vi "Format Spreadsheet Header.vi"(10 "Channel Settings":T1[](array[typedef])) -> (2 "Log file header":string)   [LabVIEW 2021, in "Logging.lvlib"]
doc: "Format a starting timestamp and column headings using the channel names from 'Channel Settings'."
uses:
  Logging.lvlib
  Acquisition/Channel Settings.ctl
  Acquisition/IO Device.ctl
  Acquisition/Sensor Type.ctl
  Acquisition/Acquisition.lvlib
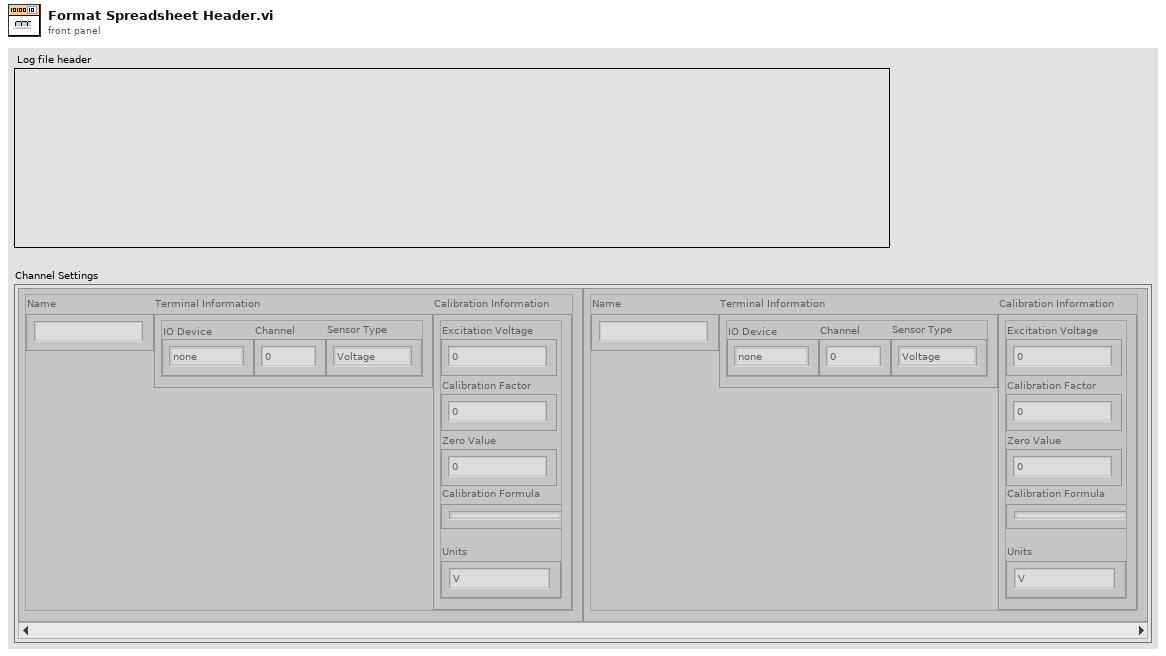
[diagram p1: front panel]
types:
  T1 = typedef "Acquisition.lvlib/Channel Settings.ctl" = cluster{"Name":string, "Terminal Information":cluster{"IO Device":T2, "Channel":i32, "Sensor Type":T3}, "Calibration Information":cluster{"Excitation Voltage":dbl, "Calibration Factor":dbl, "Zero Value":dbl, "Calibration Formula":string, "Units":string}}
  T2 = typedef "Acquisition.lvlib/IO Device.ctl" = enum16{"none", "9219", "9401"}
  T3 = typedef "Acquisition.lvlib/Sensor Type.ctl" = enum16{"Voltage", "Load", "Pressure", "Encoder"}
  T4 = cluster{"IO Device":T2, "Channel":i32, "Sensor Type":T3}
  T5 = cluster{"Excitation Voltage":dbl, "Calibration Factor":dbl, "Zero Value":dbl, "Calibration Formula":string, "Units":string}
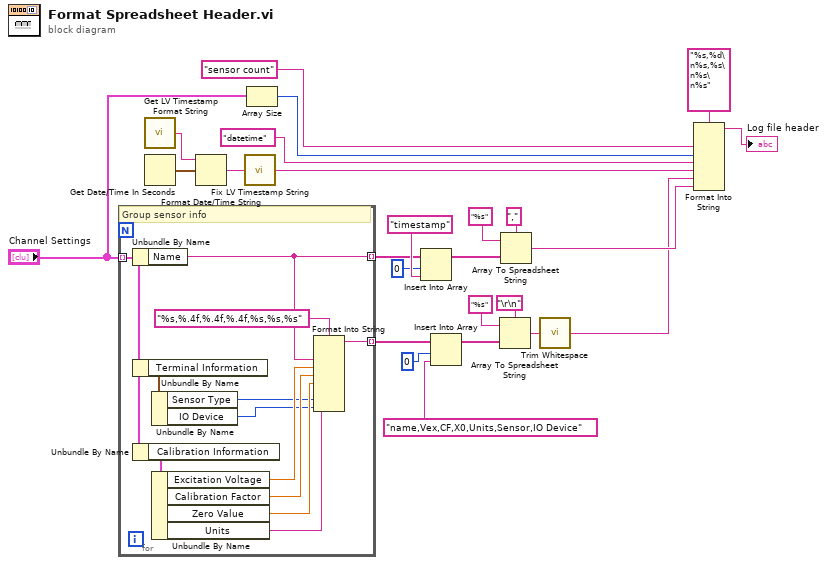
[diagram p0: block diagram]
diagram:
  n1 = for {
    tunnel: "Channel Settings" -> [w30] mode=indexing
    tunnel: [w33] -> w17 mode=indexing
    tunnel: [w32] -> w4 mode=indexing
    # "Group sensor info"
    n2 = Unbundle By Name(w30) -> ("Name"=w32:string)
    n3 = Unbundle By Name(w30) -> ("Terminal Information"=w29:T4)
    n4 = Unbundle By Name(w30) -> ("Calibration Information"=w31:T5)
    n5 = Unbundle By Name(w29) -> ("Sensor Type"=w27:T3, "IO Device"=w26:T2)
    n6 = Unbundle By Name(w31) -> ("Excitation Voltage"=w36:dbl, "Calibration Factor"=w35:dbl, "Zero Value"=w34:dbl, "Units"=w28:string)
    n7 = Format Into String(format string="%s,%.4f,%.4f,%.4f,%s,%s,%s", w32, w36, w35, w34, w28, w27, w26) -> (resulting string=w33:string)  [unwired: 2 in, 1 out]
  }
  n8 = call "Get LV Timestamp Format String.vi"() -> ("timestamp string format"=w12:string)
  n9 = Get Date/Time In Seconds() -> (seconds since 1Jan1904=w25:timestamp)
  n10 = Format Date/Time String(time format string (%c)=w12, seconds (now)=w25) -> (date/time string=w11:string)  [unwired: 1 in]
  n11 = call "Fix LV Timestamp String.vi"("LabVIEW format string"=w11) -> ("iso 8601 format string"=w8:string)
  n12 = Array Size(array="Channel Settings") -> (size(s)=w2:i32)
  n13 = Insert Into Array(array=w4, index=0, new element="timestamp" ("new element/subarray")) -> (w21:string[])
  n14 = Insert Into Array(array=w17, index=0, new element="name,Vex,CF,X0,Units,Sensor,IO Device" ("format string")) -> (w14:string[])
  n15 = Array To Spreadsheet String(delimiter (Tab)="\r\n", array=w14, 3:"%s" ("format string")) -> (spreadsheet string=w7:string)
  n16 = Array To Spreadsheet String(delimiter (Tab)=",", array=w21, 3:"%s" ("format string")) -> (spreadsheet string=w6:string)
  n17 = call <vilib>:"Trim Whitespace.vi"("string"=w7) -> ("trimmed string"=w5:string)  [unwired: 1 in]
  n18 = Format Into String(format string="%s,%d\n%s,%s\n%s\n%s", "sensor count", w2, "datetime", w8, w5, w6) -> (resulting string=→"Log file header":string)  [unwired: 2 in, 1 out]
